vi "Main Page.vi"(8 "error in (no error)":errorcluster, 11 "Node Ptr":T1 format="%.0x") -> (0 "error out":errorcluster)   [LabVIEW 2020, in "SLSC EDS System Explorer.lvlib"]
uses:
  SLSC EDS System Explorer.lvlib
  <vilib>/NI VeriStand/Custom Device API/Custom Device Item Ref.ctl
  SLSC EDS API/JSON parsing/EDSjsonStructure.ctl
  SLSC EDS API/JSON parsing/enum.ctl
  SLSC EDS API/JSON parsing/property.ctl
  SLSC EDS API/JSON parsing/command.ctl
  SLSC EDS API/JSON parsing/scale.ctl
  SLSC EDS API/JSON parsing/physicalChannel.ctl
  SLSC EDS API/JSON parsing/register.ctl
  <vilib>/Utility/error.llb/DialogType.ctl
  <vilib>/Utility/miscctls.llb/LVStringsAndValuesArrayTypeDef_U16.ctl
  Shared/Constants.vi
  <vilib>/NI VeriStand/Custom Device API/Set Item Property (Variant).vi
  <vilib>/SLSC/Initialize Session with Devices.vi
  <vilib>/SLSC/Close Session.vi
  <vilib>/NI VeriStand/Custom Device API/Custom Device API.lvlib
  Shared/SLSC EDS Shared.lvlib
  SLSC UI API/SLSC Tree Control.lvlib
  SLSC CD API/SLSC CD System Explorer/SLSC CD System Explorer.lvlib
  SLSC CD API/SLSC CD Engine/SLSC CD Engine.lvlib
  <vilib>/SLSC/SLSC.lvlib
  Engine/SLSC EDS Engine.lvlib
  SLSC EDS API/SLSC EDS API.lvlib
panel:
  out "Custom Device State":string
  in  "Refresh page":bool
  out "SLSC Device Name":string
  out "Module Name":string
  in  "Help Button":bool
  out "Slot Number":i32
  out "CD Version":string caption="Version"
  in  "Header":cluster{"Section Name":string}={"Section Name"="SLSC EDS Custom Device"}
  in  "Name":string
  in  "SHDocVw.IWebBrowser":refnum<k7>(container)
  in  "Description":string
  in  "Modify Reset Value?":bool
  in  "I8":i8
  in  "U8":u8 format="%.0x"
  in  "I32":i32
  in  "U32":u32 format="%.0x"
  in  "U64":u64 format="%.0x"
  in  "I64":i64
  in  "DBL":dbl format="%#_16g"
  in  "Ring":u16(ring)
  in  "Add":bool
  in  "Remove":bool
  in  "Header 2":cluster{"Section Name":string}={"Section Name"="Custom Device Item Settings"}
  in  "Property tree":string[](tree)
  in  "Reservation Access":i32(ring)=3 items=["None"=0, "Read Only"=1, "Read/Write"=3]
  in  "Reservation Group":string
  in  "Loop rate":u32
  in  "Apply Reset":bool
  in  "Apply Default":bool
  # "ms"
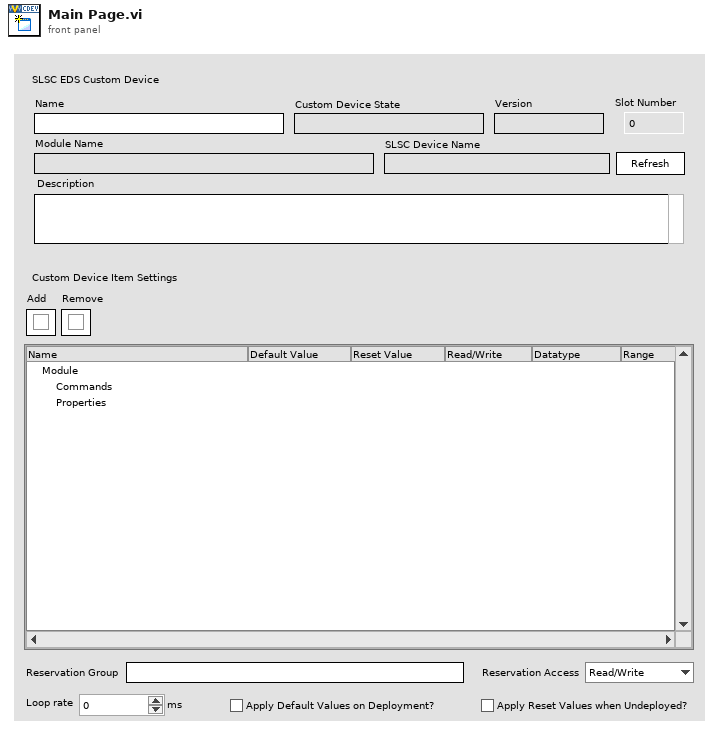
[diagram p1: front panel]
types:
  T1 = typedef "Custom Device API.lvlib/Custom Device Item Ref.ctl" = u64
  T2 = typedef "enum.ctl" = cluster{"name":string, "description-en":string, "values":cluster{"name":string, "description-en":string, "value":i32}[]}
  T3 = cluster{"Left Cell String":string, "Child Text":string[], "Child Tag":string, "Item Indent":i32, "Child Only?":bool, "Glyph Index":i32}[]
  T4 = typedef "EDSjsonStructure.ctl" = cluster{"vendorNum":u32, "vendorName":string, "vendorPrefix":string, "productNum":u32, "productName":string, "capsVersion":string, "capsSpecVersion":u32, "capsSpecOldestCompatibleVersion":u32, "enums":T2[], "properties":T5[], "commands":T6[], "scales":T7[], "physicalChannels":T8[], "registerMap":cluster{"registers":T9[]}}
  T5 = typedef "property.ctl" = cluster{"name":string, "description-en":string, "documentation-en":string, "dataType":string, "bitfield":string, "access":string, "scale":string, "value":variant, "min":variant, "max":variant, "default value":variant}
  T6 = typedef "command.ctl" = cluster{"name":string, "description-en":string, "documentation-en":string, "startBitfield":string, "waitTimeInMs":i32, "doneBitfield":string, "doneInterrupt":string, "doneTimeoutInMs":i32, "value":variant}
  T7 = typedef "scale.ctl" = cluster{"name":string, "description-en":string, "m":dbl, "b":dbl, "forwardCoeffs":dbl[], "reverseCoeffs":dbl[], "coercion":string, "table":cluster{"scaled":dbl, "unscaled":dbl}[]}
  T8 = typedef "physicalChannel.ctl" = cluster{"name":string, "description-en":string, "commands":T6[], "properties":T5[]}
  T9 = typedef "register.ctl" = cluster{"name":string, "description-en":string, "access":string, "address":u32, "size":u32, "bitfields":cluster{"name":string, "description-en":string, "offset":u32, "size":u32, "signed":bool, "strobe":bool}[]}
  T10 = typedef "LVStringsAndValuesArrayTypeDef_U16.ctl" = cluster{"String":string, "Value":u16}[]
  T11 = typedef "Custom Device API.lvlib/Custom Device Commands.ctl" = enum16{"Default", "Item renamed", "Shutdown", "Dynamic button pressed"}
  T12 = typedef "Custom Device API.lvlib/Custom Device Item Info.ctl" = cluster{"Name":string, "Is Channel":bool, "GUID":string, "Is Waveform":bool}
  T13 = typedef "DialogType.ctl" = u16
  T14 = typedef "SLSC EDS Shared.lvlib/SLSC Static Settings.ctl" = cluster{"Properties":cluster{"Boolean Properties":cluster{"property":refnum<k21>, "Value":bool, "SLSC Item":refnum<k21>, "reset value":bool}[], "Double Properties":cluster{"property":refnum<k21>, "Double Write":dbl, "SLSC Item":refnum<k21>, "Double Reset Value":dbl}[], "I32 Properties":cluster{"property":refnum<k21>, "Int32 Write":i32, "SLSC Item":refnum<k21>, "Int32 Reset Value":i32}[], "I64 Properties":cluster{"property":refnum<k21>, "Int64 Write":i64, "SLSC Item":refnum<k21>, "Int64 Reset Value":i64}[], "String Properties":cluster{"property":refnum<k21>, "String Write":string, "SLSC Item":refnum<k21>, "String Reset Value":string}[], "U32 Properties":cluster{"property":refnum<k21>, "UInt32 Write":u32, "SLSC Item":refnum<k21>, "UInt32 Reset Value":u32}[], "U64 Properties":cluster{"property":refnum<k21>, "UInt64 Write":u64, "SLSC Item":refnum<k21>, "UInt64 Reset Value":u64}[]}, "Commands":T15[], "Reset Commands":T15[], "Apply Values on Deployment":bool, "Apply Reset on Undeployment":bool, "Change Commands":T15[]}
  T15 = typedef "SLSC CD Shared.lvlib/SLSC Dynamic Channel.ctl" = cluster{"SLSC Item":string, "property":string, "Data Type":T16}
  T16 = typedef "SLSC CD Shared.lvlib/SLSC Datatype.ctl" = enum16{"Bool", "Double", "I32", "I64", "String", "U32", "U64"}
  T17 = typedef "SLSC CD Shared.lvlib/SLSC Identification.ctl" = cluster{"vendorName":string, "productNum":u32, "capsVersion":string, "capsSpecVersion":u32, "productName":string, "vendorNum":u32, "vendorPrefix":string, "capsSpecOldestCompatibleVersion":u32}
  T18 = cluster{"Left Cell String":string, "Child Text":string[], "Child Tag":string, "Item Indent":i32, "Child Only?":bool, "Glyph Index":i32}
  T19 = cluster{"name":string, "description-en":string, "value":i32}[]
  T20 = typedef "LVPoint32TypeDef.ctl" = cluster{"Horizontal":i32, "Vertical":i32}
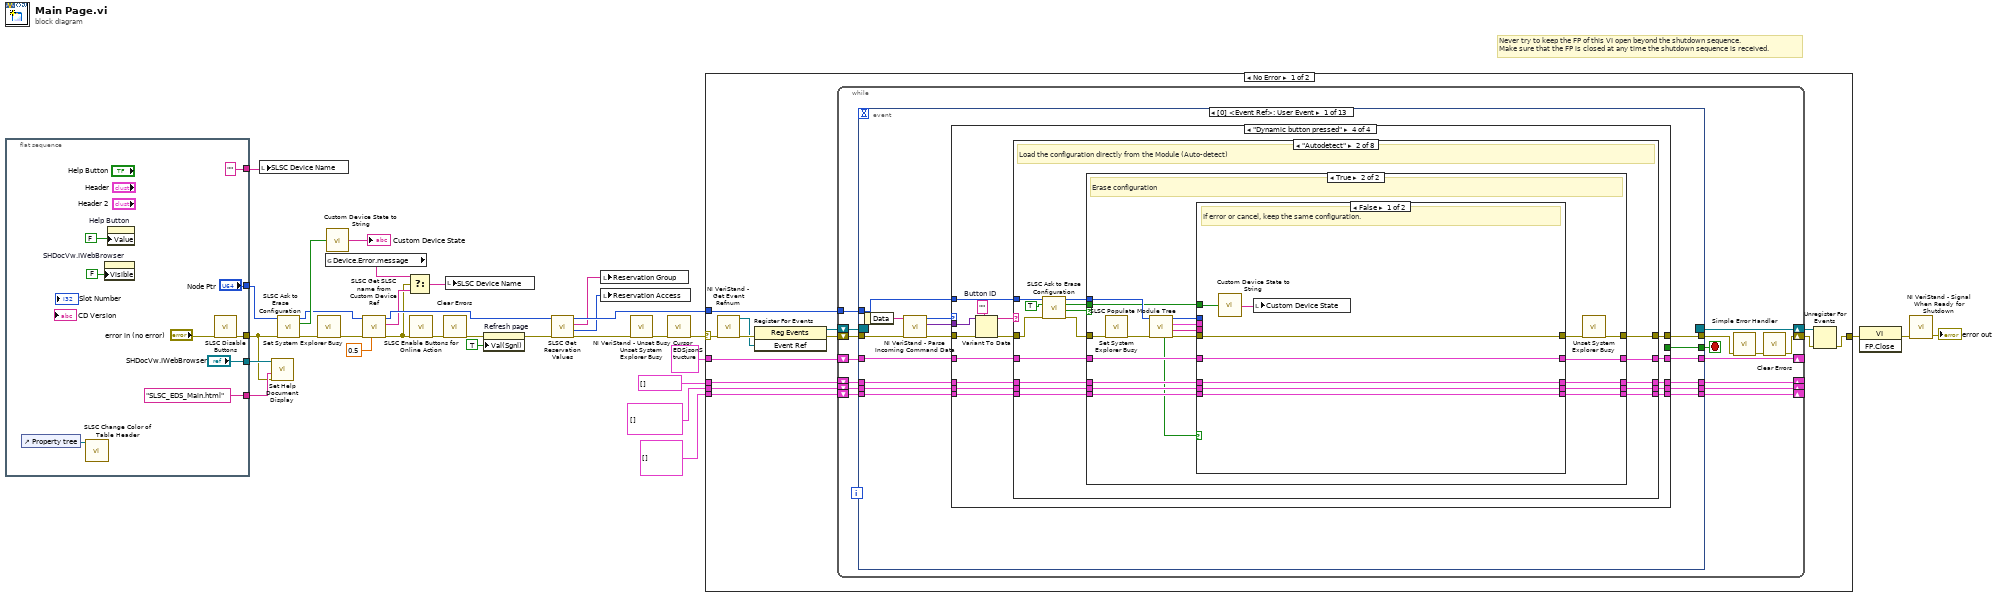
[diagram p0: block diagram]
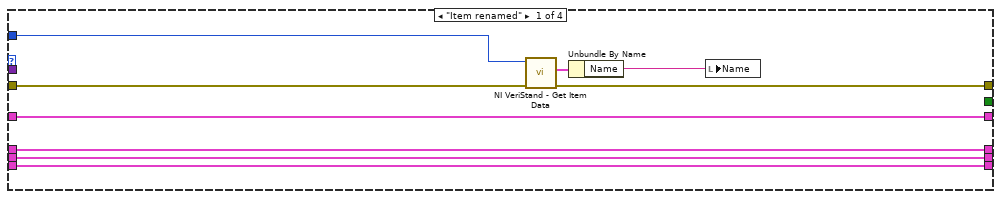
[diagram p2: hidden frame]
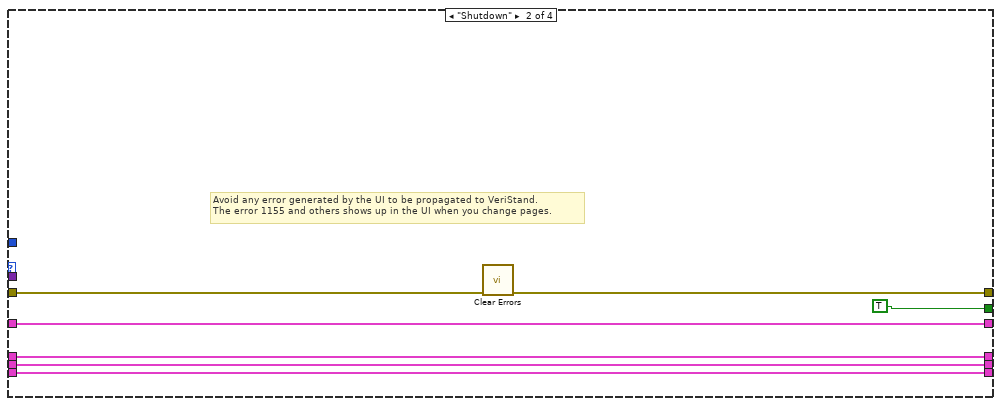
[diagram p3: hidden frame]
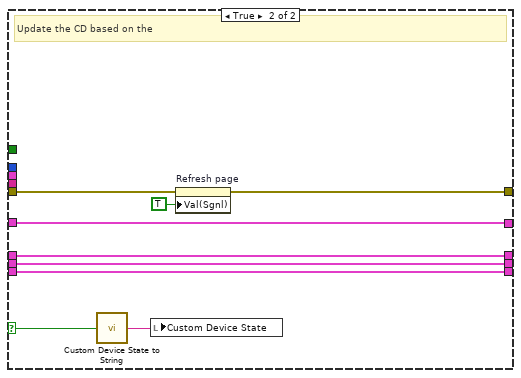
[diagram p7: hidden frame]
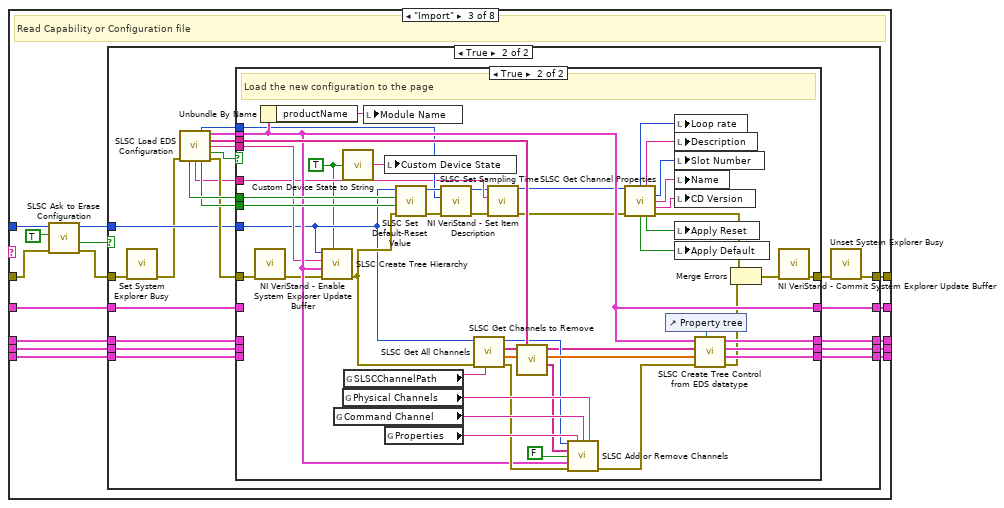
[diagram p8: hidden frame]
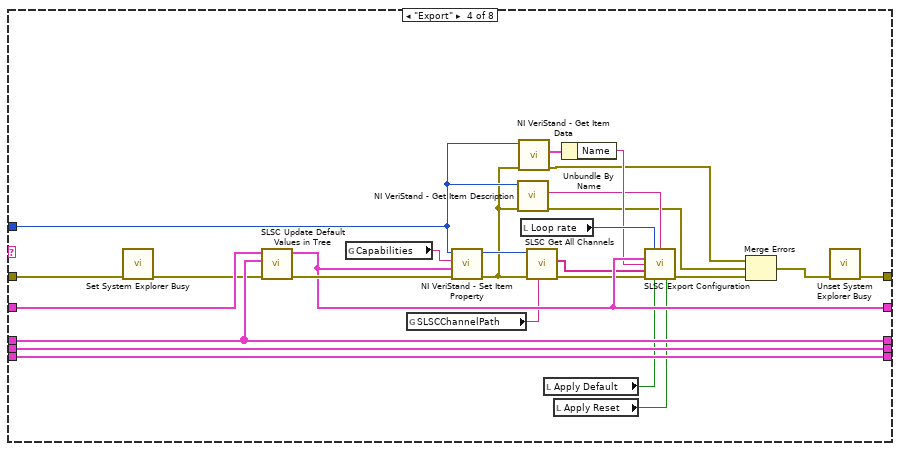
[diagram p11: hidden frame]
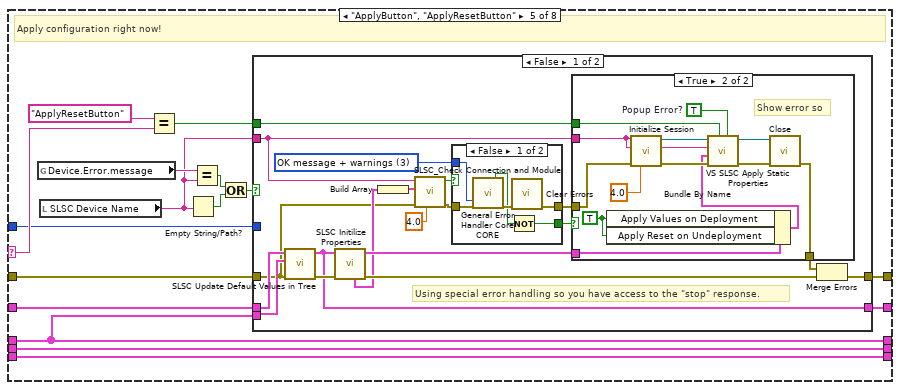
[diagram p12: hidden frame]
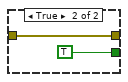
[diagram p14: hidden frame]
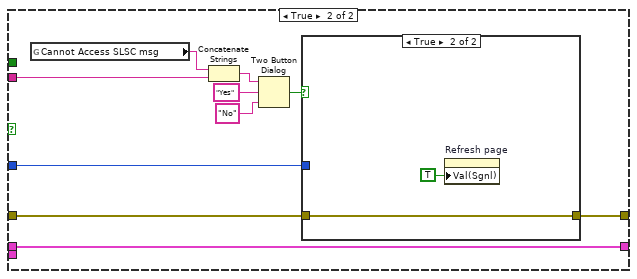
[diagram p15: hidden frame]
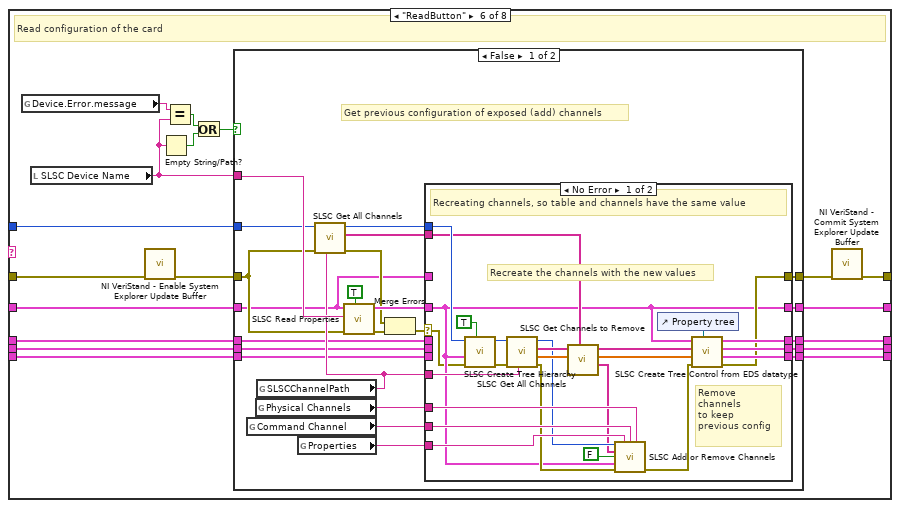
[diagram p17: hidden frame]
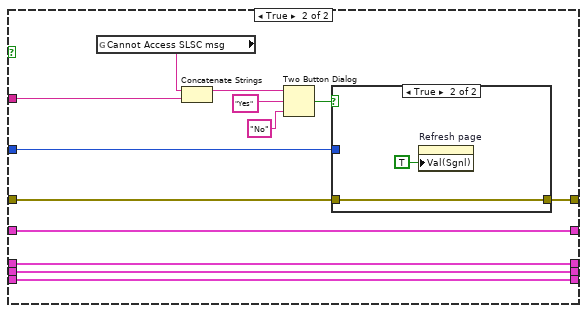
[diagram p19: hidden frame]
diagram:
  # "Never try to keep the FP of this VI open beyond the shutdown sequence.\nMake sure that the FP is closed at any time the shutdown sequence is received."
  n1 = flat-sequence {
    tunnel: ["Node Ptr"] -> w27
    tunnel: [w34] -> w28
    tunnel: ["SHDocVw.IWebBrowser"] -> w31
    tunnel: ["SLSC_EDS_Main.html" ("HTML File")] -> w30
    tunnel: ["" ("SLSC Module Name")] -> w29
    frame #0 {
      n2 = control-ref of="Property tree"() -> (w35:refnum<vi>)
      n3 = call "SLSC Change Color of Table Header.vi"("TreeControl in"=w35) -> ()  [unwired: 10 in, 1 out]
      n4 = property on="SHDocVw.IWebBrowser" class="AXCont"("Visible"=FALSE) -> ()  [unwired: 2 in, 2 out]
      n5 = property on="Help Button" class="Bool (strict)"("Value"=FALSE ("Visible")) -> ()  [unwired: 2 in, 2 out]
      n6 = call "SLSC Disable Buttons.vi"("error in (no error)"="error in (no error)") -> ("error out"=w34:errorcluster)  [unwired: 10 in]
    }
  }
  n7 = local write "SLSC Device Name"(w29) -> ()
  n8 = call "Set Help Document Display.vi"("error in (no error)"=w28, "HTML File to Load"=w30, "SHDocVw.IWebBrowser2"=w31) -> ()  [unwired: 8 in, 1 out]
  n9 = call "SLSC Ask to Erase Configuration.vi"("error in (no error)"=w28, "Device Item Ref in"=w27) -> ("error out"=w12:errorcluster, "initialized?"=w21:bool, "Item Ref out"=w10:T1)  [unwired: 6 in, 1 out]
  n10 = call "Set System Explorer Busy.vi"("error in (no error)"=w12) -> ("error out"=w11:errorcluster)  [unwired: 10 in]
  n11 = global read "Constants.vi" "Device.Error.message"() -> (w2:string)
  n12 = call "Custom Device State to String.vi"("Initialized?"=w21) -> ("Custom Device State"=→"Custom Device State":string)  [unwired: 14 in]
  n13 = call "SLSC Get SLSC name from Custom Device Ref.vi"("connect timeout"=0.5 ("connect timeout (4s)"), "error in (no error)"=w11, "Item Ref in"=w10) -> ("error out"=w4:errorcluster, "SLSC Module Name"=w5:string, "Item Ref out"=w6:T1)  [unwired: 5 in, 1 out]
  n14 = Select(t=w2, s=w4, f=w5) -> (s? t:f=w3:string)
  n15 = call "SLSC Enable Buttons for Online Action.vi"("error in (no error)"=w4) -> ("error out"=w7:errorcluster)  [unwired: 10 in]
  n16 = call <vilib>:"Clear Errors.vi"("error in (no error)"=w7) -> ("error out"=w14:errorcluster)  [unwired: 1 in, 5 out]
  n17 = local write "SLSC Device Name"(w3) -> ()
  n18 = property on="Refresh page" class="Bool (strict)"(error in=w14, "Val(Sgnl)"=TRUE ("Value (Signaling)")) -> (error out=w15:errorcluster)  [unwired: 1 in, 1 out]
  n19 = call "SLSC Get Reservation Values.vi"("Error In"=w15, "Item Ref In"=w6) -> ("Error Out"=w13:errorcluster, "Reservation Access"=w23:i32, "Reservation Group"=w24:string, "Item Ref Out"=w25:T1)  [unwired: 6 in]
  n20 = local write "Reservation Group"(w24) -> ()
  n21 = local write "Reservation Access"(w23) -> ()
  n22 = call "Unset System Explorer Busy.vi"("error in (no error)"=w13) -> ("error out"=w9:errorcluster)  [unwired: 10 in]
  n23 = call <vilib>:"NI VeriStand - Unset Busy Cursor.vi"("error in (no error)"=w9) -> ("error out"=w8:errorcluster)  [unwired: 10 in]
  n24 = case shown="No Error" w8 {
    selector: w8 -> [w47 w942]
    tunnel: [w52 w943] -> w33
    tunnel: w25 -> [w48 _]
    tunnel: T4 {"vendorNum"=0, "vendorName"="", "vendorPrefix"="", "productNum"=0, "productName"="", "capsVersion"="", "capsSpecVersion"=0, "capsSpecOldestCompatibleVersion"=1, "enums"=[], "properties"=[], "commands"=[], "scales"=[], "physicalChannels"=[], "registerMap"={"registers"=[]}} ("SLSC EDS module out") -> [w46 _]
    tunnel: T3 [] ("SLSC Output Tree") -> [w45 _]
    tunnel: T2[] [] ("Enums") -> [w44 _]
    tunnel: cluster{"name":string, string}[] [] ("Enum Strings") -> [w43 _]
    frame No Error {
      n25 = call <vilib>:"NI VeriStand - Get Event Refnum.vi"("error in (no error)"=w47) -> ("error out"=w55:errorcluster, "Event Ref"=w51:refnum<user-event>)  [unwired: 9 out]
      n26 = register-events(error in=w55, w51) -> (reference out=w49:refnum<event-registration>, error out=w50:errorcluster)  [unwired: 1 in]
      n27 = while {
        tunnel: w48 -> [w67]
        shift-right: [w65] -> w53
        shift-left: w50 -> [w70]
        shift-right: [w71] -> w54
        shift-left: w49 -> [w69]
        shift-right: [w61] -> _
        shift-left: w45 -> [w63]
        shift-right: [w59] -> _
        shift-left: w46 -> [w64]
        shift-right: [w58] -> _
        shift-left: w44 -> [w62]
        shift-right: [w57] -> _
        shift-left: w43 -> [w60]
        stop <- w68 stop-if-true
        n28 = event shown="[0] <Event Ref>: User Event" {
          selector: w69 -> [_ _ _ w802 _ _ _ _ _ _ _ _ _]
          dyn-events: [_ _ _ w802 _ _ _ _ _ _ _ _ _] -> w71
          timeout: _ -> [_ _ _ _ _ _ _ _ _ _ _ _ _]
          tunnel: w70 -> [w87 w496 w775 w795 w803 w846 w863 w870 w877 w889 w896 w898 w939]
          tunnel: [w83 _ _ _ _ _ _ _ _ _ _ _ _] -> w68
          tunnel: [w82 w496 w774 w794 w808 w813 w863 w864 w876 w888 w895 w899 w925] -> w56
          tunnel: w67 -> [w81 _ _ _ w804 w842 _ w871 w875 w887 w897 w908 w922]
          tunnel: w64 -> [w79 w495 w782 w801 w807 _ w860 w868 w878 w885 w892 w911 w931]
          tunnel: w63 -> [w78 w498 w783 w800 w810 _ w861 w872 w879 w886 w893 w916 w937]
          tunnel: w62 -> [w75 w491 w784 w797 w805 _ w858 w866 w880 w883 w890 w909 w928]
          tunnel: [w76 w498 w783 w800 w810 w827 w861 w872 w879 w886 w893 w916 w924] -> w61
          tunnel: w60 -> [w74 w492 w785 w798 w806 _ w859 w867 w881 w884 w891 w910 w929]
          tunnel: [w77 w495 w782 w801 w807 w817 w860 w868 w878 w885 w892 w911 w923] -> w59
          tunnel: [w73 w491 w784 w797 w805 w826 w858 w866 w880 w883 w890 w909 w928] -> w58
          tunnel: [w72 w492 w785 w798 w806 w825 w859 w867 w881 w884 w891 w910 w929] -> w57
          event User Event {
            n29 = event-data() -> ("Data"=w86:string)  [unwired: 1 out]
            n30 = call <vilib>:"NI VeriStand - Parse Incoming Command Data.vi"("error in (no error)"=w87, "Incoming data"=w86) -> ("error out"=w85:errorcluster, "Outgoing data"=w80:variant, "Action"=w84:T11)  [unwired: 7 out]
            n31 = case shown="\"Dynamic button pressed\"" w84 {
              tunnel: w85 -> [w96 w97 w108 w123]
              tunnel: [_ TRUE _ _] -> w83
              tunnel: [w93 w99 w108 w118] -> w82
              tunnel: w81 -> [w95 _ _ w115]
              tunnel: w80 -> [_ _ _ w122]
              tunnel: w79 -> [w91 w98 w107 w116]
              tunnel: w78 -> [w90 w102 w106 w117]
              tunnel: [w91 w98 w107 w114] -> w77
              tunnel: [w90 w102 w106 w113] -> w76
              tunnel: w75 -> [w88 w100 w104 w112]
              tunnel: w74 -> [w89 w101 w105 w111]
              tunnel: [w88 w100 w104 w110] -> w73
              tunnel: [w89 w101 w105 w109] -> w72
              frame "Item renamed" {
                n32 = call <vilib>:"NI VeriStand - Get Item Data.vi"("error in (no error)"=w96, "Item Ref in"=w95) -> ("error out"=w93:errorcluster, "Item Info"=w94:T12)  [unwired: 8 out]
                n33 = Unbundle By Name(w94) -> ("Name"=w92:string)
                n34 = local write "Name"(w92) -> ()
              }
              frame "Shutdown" {
                # "Avoid any error generated by the UI to be propagated to VeriStand.\nThe error 1155 and others shows up in the UI when you change pages."
                n35 = call <vilib>:"Clear Errors.vi"("error in (no error)"=w97) -> ("error out"=w99:errorcluster)  [unwired: 1 in, 5 out]
              }
              frame "Default", Default {
              }
              frame "Dynamic button pressed" {
                w121 = ""  # Button ID
                n36 = Variant To Data(error in=w123, type=w121, Variant=w122) -> (data=w120:string, error out=w119:errorcluster)
                n37 = case shown="\"Autodetect\"" w120 {
                  selector: w120 -> [_ _ _ _ w320 _ w467 _]
                  tunnel: w119 -> [w128 w135 w189 w301 w317 w383 w468 w484]
                  tunnel: [w128 w136 w191 w280 w316 w381 w471 w483] -> w118
                  tunnel: w117 -> [w126 w140 w195 w303 w313 w393 w465 w481]
                  tunnel: w116 -> [w127 w137 w193 w302 w321 w392 w466 w482]
                  tunnel: w115 -> [_ w134 w188 w288 w315 w391 _ _]
                  tunnel: [w127 w141 w192 w297 w314 w389 w466 w482] -> w114
                  tunnel: [w126 w142 w199 w303 w313 w388 w465 w481] -> w113
                  tunnel: w112 -> [w125 w139 w196 w298 w312 w387 w463 w479]
                  tunnel: w111 -> [w124 w138 w194 w299 w311 w386 w464 w480]
                  tunnel: [w125 w143 w198 w298 w312 w385 w463 w479] -> w110
                  tunnel: [w124 w144 w197 w299 w311 w384 w464 w480] -> w109
                  frame Default {
                  }
                  frame "Autodetect" {
                    # "Load the configuration directly from the Module (Auto-detect)"
                    n38 = call "SLSC Ask to Erase Configuration.vi"("error in (no error)"=w135, "Ask to erase?"=TRUE, "Device Item Ref in"=w134) -> ("error out"=w131:errorcluster, "Erase Data?"=w130:bool, "initialized?"=w129:bool, "Item Ref out"=w133:T1)  [unwired: 5 in]
                    n39 = case shown="True" w130 {
                      tunnel: [w147 w165] -> w144
                      tunnel: [w148 w164] -> w143
                      tunnel: [w149 w163] -> w142
                      tunnel: [w146 w162] -> w141
                      tunnel: w140 -> [w149 w160]
                      tunnel: w139 -> [w148 w159]
                      tunnel: w138 -> [w147 w158]
                      tunnel: w137 -> [w146 w157]
                      tunnel: [w145 w152] -> w136
                      tunnel: w133 -> [_ w155]
                      tunnel: w131 -> [w145 w151]
                      tunnel: w129 -> [_ w154]
                      frame False {
                        # "You decided not to erase previous configuration"
                      }
                      frame True {
                        # "Erase configuration"
                        n40 = call "Set System Explorer Busy.vi"("error in (no error)"=w151) -> ("error out"=w150:errorcluster)  [unwired: 10 in]
                        n41 = call "SLSC Populate Module Tree.vi"("error in (no error)"=w150, "Device Item Ref in"=w155) -> ("error out"=w166:errorcluster, "SLSC Module Name"=w161:string, "SLSC EDS module"=w168:T4, "Device Item Ref out"=w167:T1, "Initialized?"=w156:bool)  [unwired: 5 in]
                        n42 = case shown="False" w156 {
                          selector: w156 -> [_ w184]
                          tunnel: w168 -> [_ _]
                          tunnel: w167 -> [_ _]
                          tunnel: w166 -> [w171 w177]
                          tunnel: [w173 w179] -> w165
                          tunnel: [w174 w180] -> w164
                          tunnel: [w175 w181] -> w163
                          tunnel: [w172 w182] -> w162
                          tunnel: w161 -> [_ _]
                          tunnel: [w171 w176] -> w153
                          tunnel: w160 -> [w175 w181]
                          tunnel: w159 -> [w174 w180]
                          tunnel: w158 -> [w173 w179]
                          tunnel: w157 -> [w172 w182]
                          tunnel: w154 -> [w169 _]
                          frame False {
                            # "If error or cancel, keep the same configuration."
                            n43 = call "Custom Device State to String.vi"("Initialized?"=w169) -> ("Custom Device State"=w170:string)  [unwired: 14 in]
                            n44 = local write "Custom Device State"(w170) -> ()
                          }
                          frame True {
                            # "Update the CD based on the"
                            n45 = call "Custom Device State to String.vi"("Initialized?"=w184) -> ("Custom Device State"=w183:string)  [unwired: 14 in]
                            n46 = local write "Custom Device State"(w183) -> ()
                            n47 = property on="Refresh page" class="Bool (strict)"(error in=w177, "Val(Sgnl)"=TRUE ("Value (Signaling)")) -> (error out=w176:errorcluster)  [unwired: 1 in, 1 out]
                          }
                        }
                        n48 = call "Unset System Explorer Busy.vi"("error in (no error)"=w153) -> ("error out"=w152:errorcluster)  [unwired: 10 in]
                      }
                    }
                  }
                  frame "Import" {
                    # "Read Capability or Configuration file"
                    n49 = call "SLSC Ask to Erase Configuration.vi"("error in (no error)"=w189, "Ask to erase?"=TRUE, "Device Item Ref in"=w188) -> ("error out"=w186:errorcluster, "Erase Data?"=w185:bool, "Item Ref out"=w187:T1)  [unwired: 5 in, 1 out]
                    n50 = case shown="True" w185 {
                      tunnel: [w202 w225] -> w199
                      tunnel: [w201 w224] -> w198
                      tunnel: [w200 w223] -> w197
                      tunnel: w196 -> [w201 w222]
                      tunnel: w195 -> [w202 w215]
                      tunnel: w194 -> [w200 w214]
                      tunnel: w193 -> [w204 w213]
                      tunnel: [w204 w212] -> w192
                      tunnel: [w203 w206] -> w191
                      tunnel: w186 -> [w203 w210]
                      tunnel: w187 -> [_ w209]
                      frame False {
                        # "Decided to not overwrite previous configuration"
                      }
                      frame True {
                        n51 = call "Set System Explorer Busy.vi"("error in (no error)"=w210) -> ("error out"=w205:errorcluster)  [unwired: 10 in]
                        n52 = call "SLSC Load EDS Configuration.vi"("error in (no error)"=w205) -> ("Loop rate"=w220:u32, "SLSC EDS module out"=w226:T4, "Enable Channels"=w221:string[], "Custom Device Name"=w208:string, "Has capability?"=w216:bool, "Apply Default"=w219:bool, "Custom Device Description"=w207:string, "Apply Reset"=w218:bool, "error out"=w217:errorcluster)  [unwired: 5 in, 1 out]
                        n53 = case shown="True" w216 {
                          tunnel: w209 -> [_ w236]
                          tunnel: w226 -> [_ w251]
                          tunnel: [w231 w279] -> w225
                          tunnel: [w230 w278] -> w224
                          tunnel: [w229 w277] -> w223
                          tunnel: w222 -> [w230 _]
                          tunnel: [w228 w233] -> w211
                          tunnel: w221 -> [_ w267]
                          tunnel: w220 -> [_ w244]
                          tunnel: w219 -> [_ w262]
                          tunnel: w218 -> [_ w261]
                          tunnel: w217 -> [w228 w232]
                          tunnel: w215 -> [w231 _]
                          tunnel: w214 -> [w229 _]
                          tunnel: w213 -> [w227 _]
                          tunnel: [w227 w251] -> w212
                          tunnel: w208 -> [_ w242]
                          tunnel: w207 -> [_ w240]
                          frame False {
                            # "Error in reading the file. Don't change existent configuration."
                          }
                          frame True {
                            w234 = TRUE ("Initialized?")
                            # "Load the new configuration to the page"
                            n54 = call <vilib>:"NI VeriStand - Enable System Explorer Update Buffer.vi"("error in (no error)"=w232) -> ("error out"=w243:errorcluster)  [unwired: 10 in]
                            n55 = Unbundle By Name(w251) -> ("productName"=w263:string)
                            n56 = call "SLSC Create Tree Hierarchy.vi"("Initialized?"=w234, "error in (no error)"=w243, "SLSC EDS module"=w251, "Custom Device Name"=w242, "Item Ref in"=w236) -> ("error out"=w247:errorcluster)  [unwired: 5 in, 1 out]
                            n57 = global read "Constants.vi" "Command Channel"() -> (w272:string)
                            n58 = call "Custom Device State to String.vi"("Initialized?"=w234) -> ("Custom Device State"=w235:string)  [unwired: 14 in]
                            n59 = global read "Constants.vi" "Physical Channels"() -> (w274:string)
                            n60 = global read "Constants.vi" "SLSCChannelPath"() -> (w276:string)
                            n61 = local write "Module Name"(w263) -> ()
                            n62 = local write "Custom Device State"(w235) -> ()
                            n63 = global read "Constants.vi" "Properties"() -> (w273:string)
                            n64 = call "SLSC Set Default-Reset Value.vi"("error in (no error)"=w247, "Apply Reset"=w261, "Apply Default"=w262, "Section Ref in"=w236) -> ("error out"=w246:errorcluster, "Item Ref out"=w245:T1)  [unwired: 6 in]
                            n65 = call "SLSC Set Sampling Time.vi"("error in (no error)"=w246, "Loop rate"=w244, "Section Ref in"=w245) -> ("error out"=w241:errorcluster, "Channel Ref out"=w239:T1)  [unwired: 7 in]
                            n66 = call "SLSC Get All Channels.vi"("SLSCChannelPath"=w276, "error in (no error)"=w247, "Item Ref in"=w236) -> ("error out"=w252:errorcluster, "Channel Values"=w269:dbl[], "TreeItem Channels"=w270:string[], "Item Ref out"=w266:T1)  [unwired: 5 in]
                            n67 = call <vilib>:"NI VeriStand - Set Item Description.vi"("error in (no error)"=w241, "Description"=w240, "Item Ref in"=w239) -> ("error out"=w238:errorcluster, "Item Ref out"=w237:T1)  [unwired: 7 out]
                            n68 = call "SLSC Get Channels to Remove.vi"("Channels Created"=w267, "All Channel Values"=w269, "All Channels"=w270) -> ("Channels to be Deleted"=w265:string[], "Channel Values"=w268:dbl[], "Channels to be Added"=w264:string[])  [unwired: 6 in]
                            n69 = call "SLSC Add or Remove Channels.vi"("Section Ref in"=w266, "Properties"=w273, "Command Channel"=w272, "Physical Channels"=w274, "Property tree"=w265, "Add or Remove"=FALSE, "SLSC EDS module in"=w251, "error in (no error)"=w252) -> ("error out"=w250:errorcluster)  [unwired: 6 in, 1 out]
                            n70 = call "SLSC Get Channel Properties.vi"("Node Ptr"=w237, "error in (no error)"=w238) -> ("Loop time (ms)"=w253:u32, "Description"=w259:string, "Module Number"=w257:i32, "Name"=w260:string, "Device Version"=w256:string, "Default Value"=w255:bool, "Reset Value"=w258:bool, "error out"=w254:errorcluster)  [unwired: 5 in, 1 out]
                            n71 = control-ref of="Property tree"() -> (w275:refnum<vi>)
                            n72 = local write "Loop rate"(w253) -> ()
                            n73 = local write "Description"(w259) -> ()
                            n74 = local write "Slot Number"(w257) -> ()
                            n75 = local write "Name"(w260) -> ()
                            n76 = local write "CD Version"(w256) -> ()
                            n77 = local write "Apply Reset"(w258) -> ()
                            n78 = local write "Apply Default"(w255) -> ()
                            n79 = call "SLSC Create Tree Control from EDS datatype.vi"("Property Tree"=w275, "error in (no error)"=w250, "Channel Values"=w268, "Properties to enable"=w264, "SLSC EDS module"=w251) -> ("error out"=w249:errorcluster, "Enum Strings"=w277:cluster{"name":string, string}[], "Enums"=w278:T2[], "SLSC Output Tree"=w279:T3)  [unwired: 3 in]
                            n80 = Merge Errors(w254, w249) -> (w248:errorcluster)
                            n81 = call <vilib>:"NI VeriStand - Commit System Explorer Update Buffer.vi"("error in (no error)"=w248) -> ("error out"=w233:errorcluster)  [unwired: 10 in]
                          }
                        }
                        n82 = call "Unset System Explorer Busy.vi"("error in (no error)"=w211) -> ("error out"=w206:errorcluster)  [unwired: 10 in]
                      }
                    }
                  }
                  frame "Export" {
                    n83 = call "Set System Explorer Busy.vi"("error in (no error)"=w301) -> ("error out"=w281:errorcluster)  [unwired: 10 in]
                    n84 = call "SLSC Update Default Values in Tree.vi"("error in (no error)"=w281, "SLSC Output Tree"=w303, "SLSC EDS module in"=w302) -> ("error out"=w304:errorcluster, "SLSC EDS module out"=w297:T4)  [unwired: 7 in]
                    n85 = global read "Constants.vi" "Capabilities"() -> (w305:string)
                    n86 = global read "Constants.vi" "SLSCChannelPath"() -> (w296:string)
                    n87 = call-poly <vilib>:"NI VeriStand - Set Item Property.vi"("error in (no error)"=w304, "Value"=w297, "Property Name"=w305, "Item Ref in"=w288) -> ("error out"=w287:errorcluster, "Item Ref out"=w295:T1)  [unwired: 5 in, 1 out]
                    n88 = call <vilib>:"NI VeriStand - Get Item Description.vi"("error in (no error)"=w287, "Item Ref in"=w288) -> ("error out"=w282:errorcluster, "Description"=w285:string)  [unwired: 6 in, 2 out]
                    n89 = call <vilib>:"NI VeriStand - Get Item Data.vi"("error in (no error)"=w287, "Item Ref in"=w288) -> ("error out"=w283:errorcluster, "Item Info"=w289:T12)  [unwired: 8 out]
                    n90 = local read "Loop rate"() -> (w292:u32)
                    n91 = call "SLSC Get All Channels.vi"("SLSCChannelPath"=w296, "error in (no error)"=w287, "Item Ref in"=w295) -> ("error out"=w293:errorcluster, "TreeItem Channels"=w294:string[])  [unwired: 5 in, 2 out]
                    n92 = local read "Apply Default"() -> (w291:bool)
                    n93 = local read "Apply Reset"() -> (w290:bool)
                    n94 = Unbundle By Name(w289) -> ("Name"=w286:string)
                    n95 = call "SLSC Export Configuration.vi"("Loop rate"=w292, "Description"=w285, "SLSC EDS module in"=w297, "Custom Device Name"=w286, "Channels to Enable"=w294, "error in (no error)"=w293, "Apply Default"=w291, "Apply Reset"=w290) -> ("error out"=w300:errorcluster)  [unwired: 7 in]
                    n96 = Merge Errors(w283, w282, w300) -> (w284:errorcluster)
                    n97 = call "Unset System Explorer Busy.vi"("error in (no error)"=w284) -> ("error out"=w280:errorcluster)  [unwired: 10 in]
                  }
                  frame "ApplyButton", "ApplyResetButton" {
                    # "Apply configuration right now!"
                    n98 = global read "Constants.vi" "Device.Error.message"() -> (w309:string)
                    n99 = local read "SLSC Device Name"() -> (w307:string)
                    n100 = Equal?(x="ApplyResetButton", y=w320) -> (x = y?=w319:bool)
                    n101 = Empty String/Path?(string/path=w307) -> (empty?=w310:bool)
                    n102 = Equal?(x=w309, y=w307) -> (x = y?=w308:bool)
                    n103 = Or(x=w308, y=w310) -> (x .or. y?=w306:bool)
                    n104 = case shown="False" w306 {
                      tunnel: w313 -> [w340 _]
                      tunnel: w321 -> [w332 w366]
                      tunnel: w319 -> [w339 _]
                      tunnel: w317 -> [w327 w371]
                      tunnel: [w337 w367] -> w316
                      tunnel: w307 -> [w331 w372]
                      tunnel: w315 -> [_ w370]
                      tunnel: [w333 w366] -> w314
                      frame False {
                        w322 = T13 3 items=["no dialog", "OK message", "continue or stop message", "OK message + warnings", "continue/stop + warnings"] ("type of dialog (OK msg:1)")
                        # "Using special error handling so you have access to the \"stop\" response."
                        n105 = call "SLSC Update Default Values in Tree.vi"("error in (no error)"=w327, "SLSC Output Tree"=w340, "SLSC EDS module in"=w332) -> ("error out"=w338:errorcluster, "SLSC EDS module out"=w333:T4)  [unwired: 7 in]
                        n106 = call "SLSC Initilize Properties.vi"("error in (no error)"=w338, "Capabilities"=w333) -> ("error out"=w336:errorcluster, "Configuration Data"=w335:T14, "Identification"=w330:T17)  [unwired: 5 in, 2 out]
                        n107 = Build Array(w330) -> (w329:T17[])
                        n108 = call "SLSC_Check Connection and Module.vi"("Connect timeout (s)"=4.0 ("connect timeout (10 sec)"), "error in (no error)"=w327, "Supported Modules"=w329, "devices"=w331) -> ("error out"=w325:errorcluster, "Device Found?"=w326:bool)  [unwired: 6 in]
                        n109 = case shown="False" w326 {
                          tunnel: [w355 TRUE ("T button?")] -> w324
                          tunnel: w325 -> [w359 w361]
                          tunnel: [w360 w361] -> w323
                          tunnel: w322 -> [w357 _]
                          frame False {
                            n110 = call <vilib>:"General Error Handler Core CORE.vi"("type of dialog (OK msg:1)"=w357, "error in (no error)"=w359) -> ("stop event propagated"=w356:bool, "error out"=w358:errorcluster)  [unwired: 12 in, 4 out]
                            n111 = Not(x=w356) -> (.not. x?=w355:bool)
                            n112 = call <vilib>:"Clear Errors.vi"("error in (no error)"=w358) -> ("error out"=w360:errorcluster)  [unwired: 5 in, 1 out]
                          }
                          frame True {
                          }
                        }
                        n113 = case shown="True" w324 {
                          tunnel: w339 -> [_ w349]
                          tunnel: w335 -> [_ w347]
                          tunnel: [w341 w344] -> w334
                          tunnel: w331 -> [_ w343]
                          tunnel: w323 -> [w341 w342]
                          frame False {
                            # "Avoid messaging incorrect board.\nAnd we ask just in case the user is \nsure the board is correct, just happen\nto not match the Board number"
                          }
                          frame True {
                            w345 = TRUE ("Apply Values on Deployment")
                            w348 = TRUE  # Popup Error?
                            # "Show error so"
                            n114 = Bundle By Name(cluster=w347, "Apply Values on Deployment"=w345, "Apply Reset on Undeployment"=w345) -> (w346:T14)
                            n115 = call-poly <vilib>:"Initialize Session.vi"("devices"=w343, "error in (no error)"=w342, "connect timeout (60 sec)"=4.0 ("connect timeout (10 sec)")) -> ("session out"=w353:refnum<k21>, "error out"=w354:errorcluster)  [unwired: 11 in]
                            n116 = call "VS SLSC Apply Static Properties.vi"("Popup Error?"=w348, "Reset?"=w349, "error in (no error)"=w354, "Configuration Data"=w346, "SLSC Module Name in"=w343, "Refnum in"=w353) -> ("error out"=w351:errorcluster, "Refnum out"=w350:refnum<k21>)  [unwired: 3 in, 1 out]
                            n117 = call-poly <vilib>:"Close.vi"("session in"=w350, "error in (no error)"=w351) -> ("error out"=w344:errorcluster)  [unwired: 13 in]
                          }
                        }
                        n118 = Merge Errors(w334, w336) -> (w337:errorcluster)
                      }
                      frame True {
                        n119 = global read "Constants.vi" "Cannot Access SLSC msg"() -> (w364:string)
                        n120 = Concatenate Strings(w364, w372) -> (w369:string)
                        n121 = Two Button Dialog(message=w369, 1:"No" ("F button name (\"Cancel\")"), 2:"Yes" ("F button name (\"Cancel\")")) -> (T button?=w368:bool)
                        n122 = case shown="True" w368 {
                          tunnel: w371 -> [w373 w375]
                          tunnel: w370 -> [_ _]
                          tunnel: [w373 w375] -> w367
                          frame False {
                          }
                          frame True {
                            n123 = property on="Refresh page" class="Bool (strict)"("Val(Sgnl)"=TRUE ("Value (Signaling)")) -> ()  [unwired: 2 in, 2 out]
                          }
                        }
                      }
                    }
                  }
                  frame "ReadButton" {
                    # "Read configuration of the card"
                    n124 = global read "Constants.vi" "Device.Error.message"() -> (w378:string)
                    n125 = local read "SLSC Device Name"() -> (w377:string)
                    n126 = call <vilib>:"NI VeriStand - Enable System Explorer Update Buffer.vi"("error in (no error)"=w383) -> ("error out"=w382:errorcluster)  [unwired: 10 in]
                    n127 = Empty String/Path?(string/path=w377) -> (empty?=w390:bool)
                    n128 = Equal?(x=w378, y=w377) -> (x = y?=w376:bool)
                    n129 = Or(x=w376, y=w390) -> (x .or. y?=w379:bool)
                    n130 = case shown="False" w379 {
                      tunnel: w393 -> [w397 w452]
                      tunnel: w392 -> [w398 w453]
                      tunnel: w382 -> [w404 w458]
                      tunnel: [w401 w454] -> w380
                      tunnel: w377 -> [w416 w459]
                      tunnel: w391 -> [w411 w457]
                      tunnel: [w399 w453] -> w389
                      tunnel: [w415 w452] -> w388
                      tunnel: w387 -> [w396 w450]
                      tunnel: w386 -> [w395 w449]
                      tunnel: [w407 w450] -> w385
                      tunnel: [w406 w449] -> w384
                      frame False {
                        # "Get previous configuration of exposed (add) channels"
                        n131 = global read "Constants.vi" "Command Channel"() -> (w412:string)
                        n132 = global read "Constants.vi" "Physical Channels"() -> (w414:string)
                        n133 = global read "Constants.vi" "SLSCChannelPath"() -> (w410:string)
                        n134 = global read "Constants.vi" "Properties"() -> (w413:string)
                        n135 = call "SLSC Get All Channels.vi"("SLSCChannelPath"=w410, "error in (no error)"=w404, "Item Ref in"=w411) -> ("error out"=w402:errorcluster, "TreeItem Channels"=w408:string[], "Item Ref out"=w409:T1)  [unwired: 5 in, 1 out]
                        n136 = call "SLSC Read Properties.vi"("Default Only?"=TRUE ("Read Only?"), "error in (no error)"=w404, "SLSC Device"=w416, "SLSC EDS module in"=w398) -> ("error out"=w403:errorcluster, "SLSC EDS module out"=w405:T4)  [unwired: 6 in]
                        n137 = Merge Errors(w402, w403) -> (w400:errorcluster)
                        n138 = case shown="No Error" w400 {
                          selector: w400 -> [w417 w445]
                          tunnel: [w441 w444] -> w415
                          tunnel: w414 -> [w438 _]
                          tunnel: w413 -> [w437 _]
                          tunnel: w412 -> [w436 _]
                          tunnel: w410 -> [w430 _]
                          tunnel: w409 -> [w429 _]
                          tunnel: w408 -> [w428 _]
                          tunnel: [w423 w443] -> w407
                          tunnel: [w422 w442] -> w406
                          tunnel: w405 -> [w418 _]
                          tunnel: [w419 w445] -> w401
                          tunnel: [w418 w446] -> w399
                          tunnel: w398 -> [_ w446]
                          tunnel: w397 -> [_ w444]
                          tunnel: w396 -> [_ w443]
                          tunnel: w395 -> [_ w442]
                          frame No Error {
                            # "Remove \nchannels\nto keep \nprevious config"
                            # "Recreate the channels with the new values"
                            # "Recreating channels, so table and channels have the same value"
                            n139 = call "SLSC Create Tree Hierarchy.vi"("Initialized?"=TRUE, "error in (no error)"=w417, "SLSC EDS module"=w418, "Item Ref in"=w429) -> ("error out"=w434:errorcluster, "Parent Ref out"=w433:T1)  [unwired: 6 in]
                            n140 = call "SLSC Get All Channels.vi"("SLSCChannelPath"=w430, "error in (no error)"=w434, "Item Ref in"=w433) -> ("error out"=w421:errorcluster, "Channel Values"=w431:dbl[], "TreeItem Channels"=w432:string[], "Item Ref out"=w426:T1)  [unwired: 5 in]
                            n141 = call "SLSC Get Channels to Remove.vi"("Channels Created"=w428, "All Channel Values"=w431, "All Channels"=w432) -> ("Channels to be Deleted"=w425:string[], "Channel Values"=w427:dbl[], "Channels to be Added"=w424:string[])  [unwired: 6 in]
                            n142 = call "SLSC Add or Remove Channels.vi"("Section Ref in"=w426, "Properties"=w437, "Command Channel"=w436, "Physical Channels"=w438, "Property tree"=w425, "Add or Remove"=FALSE, "SLSC EDS module in"=w418, "error in (no error)"=w421) -> ("error out"=w420:errorcluster)  [unwired: 6 in, 1 out]
                            n143 = control-ref of="Property tree"() -> (w440:refnum<vi>)
                            n144 = call "SLSC Create Tree Control from EDS datatype.vi"("Property Tree"=w440, "error in (no error)"=w420, "Channel Values"=w427, "Properties to enable"=w424, "SLSC EDS module"=w418) -> ("error out"=w419:errorcluster, "Enum Strings"=w422:cluster{"name":string, string}[], "Enums"=w423:T2[], "SLSC Output Tree"=w441:T3)  [unwired: 3 in]
                          }
                          frame Error {
                            # "If error, don't change state and report the error (outside)"
                          }
                        }
                      }
                      frame True {
                        n145 = global read "Constants.vi" "Cannot Access SLSC msg"() -> (w448:string)
                        n146 = Concatenate Strings(w448, w459) -> (w456:string)
                        n147 = Two Button Dialog(message=w456, 1:"No" ("F button name (\"Cancel\")"), 2:"Yes" ("F button name (\"Cancel\")")) -> (T button?=w455:bool)
                        n148 = case shown="True" w455 {
                          tunnel: w458 -> [w460 w462]
                          tunnel: w457 -> [_ _]
                          tunnel: [w460 w462] -> w454
                          frame False {
                          }
                          frame True {
                            n149 = property on="Refresh page" class="Bool (strict)"("Val(Sgnl)"=TRUE ("Value (Signaling)")) -> ()  [unwired: 2 in, 2 out]
                          }
                        }
                      }
                    }
                    n150 = call <vilib>:"NI VeriStand - Commit System Explorer Update Buffer.vi"("error in (no error)"=w380) -> ("error out"=w381:errorcluster)  [unwired: 10 in]
                  }
                  frame "Diagram", "Pinout" {
                    # "Open and forget..."
                    n151 = vi-ref "SLSC Show Pinout.vi"() -> (w469:refnum<vi>)
                    n152 = property class="VI Interface Type 1"(reference=w469) -> ("Name"=w470:string)  [unwired: 1 in, 2 out]
                    n153 = Unbundle By Name(w466) -> ("vendorPrefix"=w476:string, "productNum"=w475:u32)
                    n154 = Open VI Reference(type specifier VI Refnum (for type only)=w469, vi path=w470, options=128, error in (no error)=w468) -> (vi reference=w477:refnum<vi>, error out=w473:errorcluster)  [unwired: 2 in]
                    n155 = call-by-ref "Start Asynchronous Call"(reference=w477, error in=w473, "Type"=w467, "number"=w475, "Vendor Name"=w476) -> (reference out=w474:refnum<vi>, error out=w472:errorcluster)  [unwired: 9 in]
                    n156 = Close Reference(reference=w474, error in (no error)=w472) -> (error out=w471:errorcluster)
                  }
                  frame "HelpButton" {
                    # "Show Help Page"
                    n157 = property on="SHDocVw.IWebBrowser" class="AXCont"(error in=w484) -> (error out=w485:errorcluster, "Visible"=w487:bool)  [unwired: 1 in, 1 out]
                    n158 = Not(x=w487) -> (.not. x?=w486:bool)
                    n159 = property on="SHDocVw.IWebBrowser" class="AXCont"(error in=w485, "Visible"=w486) -> (error out=w483:errorcluster)  [unwired: 1 in, 1 out]
                  }
                }
              }
            }
          }
          event "Property tree": Value Change {
            n160 = event-data() -> ()  [unwired: 2 out]
            n161 = control-ref of="Modify Reset Value?"() -> (w497:refnum<vi>)
            n162 = control-ref of="DBL"() -> (w506:refnum<vi>)
            n163 = control-ref of="I8"() -> (w504:refnum<vi>)
            n164 = control-ref of="I32"() -> (w499:refnum<vi>)
            n165 = control-ref of="I64"() -> (w500:refnum<vi>)
            n166 = control-ref of="U8"() -> (w501:refnum<vi>)
            n167 = control-ref of="U32"() -> (w502:refnum<vi>)
            n168 = control-ref of="U64"() -> (w503:refnum<vi>)
            n169 = control-ref of="Ring"() -> (w505:refnum<vi>)
            n170 = Array Size(array="Property tree") -> (size(s)=w494:i32)
            n171 = Equal To 0?(x=w494) -> (x = 0?=w489:bool)
            n172 = Not Equal?(x=w494, y=1 ("x")) -> (x != y?=w493:bool)
            n173 = case shown="False" w489 {
              tunnel: "Property tree" -> [w512 _]
              tunnel: w498 -> [w513 _]
              tunnel: w491 -> [w522 _]
              tunnel: w503 -> [w523 w764]
              tunnel: w502 -> [w529 w765]
              tunnel: w501 -> [w524 w766]
              tunnel: w500 -> [w525 w767]
              tunnel: w499 -> [w526 w768]
              tunnel: w504 -> [w527 w769]
              tunnel: w505 -> [w530 w770]
              tunnel: w506 -> [w528 w771]
              tunnel: w492 -> [w519 _]
              tunnel: "Modify Reset Value?" -> [w515 _]
              tunnel: w497 -> [w516 w762]
              tunnel: w493 -> [w514 _]
              frame False {
                # "Use the default control based on the first selection"
                # "Only allow to modify the value of 1 selection, otherwise hide control."
                n174 = Index Array(array=w512) -> (element=w521:string)  [unwired: 1 in]
                n175 = call "SLSC Search Item in Tree Control.vi"("SLSC Output Tree"=w513, "Item Tag"=w521) -> ("Item"=w520:T18)  [unwired: 10 in, 3 out]
                n176 = call "SLSC Get Items from Tree Control.vi"("Item"=w520) -> ("Value"=w511:string, "Datatype"=w508:string, "Type of Channel"=w510:string, "Reset Value"=w517:string)  [unwired: 6 in, 1 out]
                n177 = case shown="True" w514 {
                  tunnel: w513 -> [_ w539]
                  tunnel: w512 -> [_ w538]
                  tunnel: w508 -> [_ w537]
                  tunnel: w510 -> [w531 w535]
                  tunnel: [w531 w534] -> w509
                  frame False {
                  }
                  frame True {
                    n178 = for {
                      tunnel: w539 -> [w549]
                      tunnel: w538 -> [w547] mode=indexing
                      tunnel: w537 -> [w546]
                      tunnel: [w545] -> w536 mode=indexing
                      tunnel: w535 -> [w542]
                      stop <- w545 continue-if-true
                      n179 = call "SLSC Search Item in Tree Control.vi"("SLSC Output Tree"=w549, "Item Tag"=w547) -> ("Item"=w548:T18)  [unwired: 10 in, 3 out]
                      n180 = call "SLSC Get Items from Tree Control.vi"("Item"=w548) -> ("Datatype"=w540:string, "Type of Channel"=w543:string)  [unwired: 6 in, 3 out]
                      n181 = Equal?(x=w542, y=w543) -> (x = y?=w541:bool)
                      n182 = Equal?(x=w540, y=w546) -> (x = y?=w544:bool)
                      n183 = And(x=w541, y=w544) -> (x .and. y?=w545:bool)
                    }
                    n184 = And Array Elements(Boolean array=w536) -> (logical AND=w532:bool)
                    n185 = Select(t=w535, s=w532, f="Diff" ("t")) -> (s? t:f=w534:string)
                  }
                }
                n186 = Select(t=w517, s=w515, f=w511) -> (s? t:f=w518:string)
                n187 = case shown="Default" w509 {
                  tunnel: w508 -> [w563 _]
                  tunnel: w530 -> [w562 w758]
                  tunnel: w529 -> [w561 w753]
                  tunnel: w528 -> [w560 w759]
                  tunnel: w527 -> [w559 w757]
                  tunnel: w526 -> [w558 w756]
                  tunnel: w525 -> [w557 w755]
                  tunnel: w524 -> [w556 w754]
                  tunnel: w523 -> [w555 w751]
                  tunnel: w522 -> [w554 _]
                  tunnel: w518 -> [w553 _]
                  tunnel: w519 -> [w552 _]
                  tunnel: w516 -> [w551 w750]
                  tunnel: w515 -> [w550 _]
                  frame Default {
                    # "Show the type of control for Writing"
                    n188 = case shown="\"U32\", \"UInt32\"" w563 {
                      selector: w563 -> [w568 w586 w602 w618 w634 w647 w668 w686 w704 w734]
                      tunnel: w562 -> [w572 w594 w610 w626 w641 w660 w678 w695 w703 w733]
                      tunnel: w561 -> [w571 w591 w605 w622 w643 w655 w672 w689 w709 w738]
                      tunnel: w560 -> [w579 w595 w611 w627 w642 w661 w679 w688 w714 w743]
                      tunnel: w559 -> [w578 w587 w609 w625 w640 w659 w677 w694 w713 w742]
                      tunnel: w558 -> [w577 w589 w603 w620 w639 w658 w676 w693 w712 w741]
                      tunnel: w557 -> [w576 w593 w608 w624 w638 w653 w675 w692 w711 w740]
                      tunnel: w556 -> [w575 w588 w607 w619 w637 w657 w674 w691 w710 w739]
                      tunnel: w555 -> [w574 w590 w604 w621 w636 w654 w671 w687 w708 w737]
                      tunnel: w554 -> [_ _ _ _ _ _ _ _ w715 _]
                      tunnel: w553 -> [w567 w585 w601 w617 w633 w646 w667 w685 w706 w735]
                      tunnel: w552 -> [_ _ _ _ _ _ _ _ w705 _]
                      tunnel: w551 -> [w564 w583 w599 w615 w631 w649 w665 w683 w699 w729]
                      tunnel: w550 -> [_ _ _ _ _ _ _ _ _ w725]
                      frame "Bool", "Boolean" {
                        w565 = TRUE ("Visible")
                        n189 = call "SLSC Convert Items - String to Variants.vi"("Datatype"=w568, "Value"=w567) -> ("Value (DBL)"=w566:dbl)  [unwired: 10 in, 3 out]
                        n190 = Build Array(w579, w571, w578, w577, w576, w575, w574) -> (w573:refnum<vi>[])
                        n191 = for {
                          tunnel: w573 -> [w581] mode=indexing
                          n192 = property class="DigNum"(reference=w581, "Visible"=FALSE) -> ()  [unwired: 1 in, 2 out]
                        }
                        n193 = property on="Ring" class="Ring (strict)"("StringsAndValues[]"=T10 [{"String"="False", "Value"=0}, {"String"="True", "Value"=1}] ("Strings And Values []")) -> (error out=w569:errorcluster)  [unwired: 2 in, 1 out]
                        n194 = property class="Ring (strict)"(reference=w572, error in=w569, "Visible"=w565, "Value"=w566) -> ()  [unwired: 2 out]
                        n195 = property class="Bool (strict)"(reference=w564, "Visible"=w565) -> ()  [unwired: 1 in, 2 out]
                      }
                      frame "I8", "Int8" {
                        w582 = TRUE ("Visible")
                        n196 = call "SLSC Convert Items - String to Variants.vi"("Datatype"=w586, "Value"=w585) -> ("Value (DBL)"=w584:dbl)  [unwired: 10 in, 3 out]
                        n197 = Build Array(w595, w594, w588, w590, w593, w589, w591) -> (w592:refnum<vi>[])
                        n198 = for {
                          tunnel: w592 -> [w597] mode=indexing
                          n199 = property class="Num"(reference=w597, "Visible"=FALSE) -> ()  [unwired: 1 in, 2 out]
                        }
                        n200 = property class="DigNum (strict)"(reference=w587, "Visible"=w582, "Value"=w584) -> ()  [unwired: 1 in, 2 out]
                        n201 = property class="Bool (strict)"(reference=w583, "Visible"=w582) -> ()  [unwired: 1 in, 2 out]
                      }
                      frame "I32", "Int32" {
                        w598 = TRUE ("Visible")
                        n202 = call "SLSC Convert Items - String to Variants.vi"("Datatype"=w602, "Value"=w601) -> ("Value (DBL)"=w600:dbl)  [unwired: 10 in, 3 out]
                        n203 = Build Array(w611, w610, w609, w604, w608, w607, w605) -> (w606:refnum<vi>[])
                        n204 = for {
                          tunnel: w606 -> [w613] mode=indexing
                          n205 = property class="Num"(reference=w613, "Visible"=FALSE) -> ()  [unwired: 1 in, 2 out]
                        }
                        n206 = property class="DigNum (strict)"(reference=w603, "Visible"=w598, "Value"=w600) -> ()  [unwired: 1 in, 2 out]
                        n207 = property class="Bool (strict)"(reference=w599, "Visible"=w598) -> ()  [unwired: 1 in, 2 out]
                      }
                      frame "U8", "UInt8" {
                        w614 = TRUE ("Visible")
                        n208 = call "SLSC Convert Items - String to Variants.vi"("Datatype"=w618, "Value"=w617) -> ("Value (DBL)"=w616:dbl)  [unwired: 10 in, 3 out]
                        n209 = Build Array(w627, w626, w625, w621, w624, w620, w622) -> (w623:refnum<vi>[])
                        n210 = for {
                          tunnel: w623 -> [w629] mode=indexing
                          n211 = property class="Num"(reference=w629, "Visible"=FALSE) -> ()  [unwired: 1 in, 2 out]
                        }
                        n212 = property class="DigNum (strict)"(reference=w619, "Visible"=w614, "Value"=w616) -> ()  [unwired: 1 in, 2 out]
                        n213 = property class="Bool (strict)"(reference=w615, "Visible"=w614) -> ()  [unwired: 1 in, 2 out]
                      }
                      frame "U32", "UInt32" {
                        w630 = TRUE ("Visible")
                        n214 = Build Array(w642, w641, w640, w639, w638, w637, w636) -> (w635:refnum<vi>[])
                        n215 = call "SLSC Convert Items - String to Variants.vi"("Datatype"=w634, "Value"=w633) -> ("Value (DBL)"=w632:dbl)  [unwired: 10 in, 3 out]
                        n216 = for {
                          tunnel: w635 -> [w645] mode=indexing
                          n217 = property class="Num"(reference=w645, "Visible"=FALSE) -> ()  [unwired: 1 in, 2 out]
                        }
                        n218 = property class="DigNum (strict)"(reference=w643, "Visible"=w630, "Value"=w632) -> ()  [unwired: 1 in, 2 out]
                        n219 = property class="Bool (strict)"(reference=w631, "Visible"=w630) -> ()  [unwired: 1 in, 2 out]
                      }
                      frame "I64", "Int64" {
                        w648 = TRUE ("Visible")
                        n220 = call "SLSC Convert Items - String to Variants.vi"("Datatype"=w647, "Value"=w646) -> ("Value"=w652:variant)  [unwired: 10 in, 3 out]
                        n221 = Build Array(w661, w660, w659, w658, w654, w657, w655) -> (w656:refnum<vi>[])
                        n222 = for {
                          tunnel: w656 -> [w663] mode=indexing
                          n223 = property class="Num"(reference=w663, "Visible"=FALSE) -> ()  [unwired: 1 in, 2 out]
                        }
                        n224 = Variant To Data(type=i64 0, Variant=w652) -> (data=w650:i64)  [unwired: 1 in, 1 out]
                        n225 = property class="DigNum (strict)"(reference=w653, "Visible"=w648, "Value"=w650) -> ()  [unwired: 1 in, 2 out]
                        n226 = property class="Bool (strict)"(reference=w649, "Visible"=w648) -> ()  [unwired: 1 in, 2 out]
                      }
                      frame "U64", "UInt64" {
                        w664 = TRUE ("Visible")
                        n227 = call "SLSC Convert Items - String to Variants.vi"("Datatype"=w668, "Value"=w667) -> ("Value"=w666:variant)  [unwired: 10 in, 3 out]
                        n228 = Build Array(w679, w678, w677, w676, w675, w674, w672) -> (w673:refnum<vi>[])
                        n229 = for {
                          tunnel: w673 -> [w681] mode=indexing
                          n230 = property class="Num"(reference=w681, "Visible"=FALSE) -> ()  [unwired: 1 in, 2 out]
                        }
                        n231 = Variant To Data(type=u64 0, Variant=w666) -> (data=w669:u64)  [unwired: 1 in, 1 out]
                        n232 = property class="Bool (strict)"(reference=w665, "Visible"=w664) -> ()  [unwired: 1 in, 2 out]
                        n233 = property class="DigNum (strict)"(reference=w671, "Visible"=w664, "Value"=w669) -> ()  [unwired: 1 in, 2 out]
                      }
                      frame "DBL", "Double" {
                        w682 = TRUE ("Visible")
                        n234 = call "SLSC Convert Items - String to Variants.vi"("Datatype"=w686, "Value"=w685) -> ("Value (DBL)"=w684:dbl)  [unwired: 10 in, 3 out]
                        n235 = Build Array(w687, w695, w694, w693, w692, w691, w689) -> (w690:refnum<vi>[])
                        n236 = for {
                          tunnel: w690 -> [w697] mode=indexing
                          n237 = property class="Num"(reference=w697, "Visible"=FALSE) -> ()  [unwired: 1 in, 2 out]
                        }
                        n238 = property class="DigNum (strict)"(reference=w688, "Visible"=w682, "Value"=w684) -> ()  [unwired: 1 in, 2 out]
                        n239 = property class="Bool (strict)"(reference=w683, "Visible"=w682) -> ()  [unwired: 1 in, 2 out]
                      }
                      frame Default {
                        n240 = Build Array(w714, w713, w712, w711, w710, w709, w708) -> (w707:refnum<vi>[])
                        n241 = call "SLSC Search and Convert ENUM Value by Name.vi"("Enum Strings"=w705, "enums"=w715, "Value"=w706, "Datatype Name"=w704) -> ("Enum"=w701:T2, "Datatype found?"=w698:bool, "Value"=w702:i32)  [unwired: 5 in]
                        n242 = for {
                          tunnel: w707 -> [w717] mode=indexing
                          n243 = property class="DigNum"(reference=w717, "Visible"=FALSE) -> ()  [unwired: 1 in, 2 out]
                        }
                        n244 = case shown="False" w698 {
                          tunnel: w701 -> [_ w720]
                          frame False {
                            # "Datatype not found: hide all controls"
                          }
                          frame True {
                            # "Show Ring control for custom datatype"
                            n245 = Unbundle By Name(w720) -> ("values"=w719:T19)
                            n246 = for {
                              tunnel: w719 -> [w724] mode=indexing
                              tunnel: [w721] -> w718 mode=indexing
                              n247 = Unbundle(w724) -> ("name"=w723:string, "value"=w722:i32)  [unwired: 1 out]
                              n248 = Bundle("name"=w723, "value"=w722) -> (w721:cluster{"name":string, "value":i32})  [unwired: 1 in]
                            }
                            n249 = property on="Ring" class="Ring (strict)"("StringsAndValues[]"=w718) -> ()  [unwired: 2 in, 2 out]
                          }
                        }
                        n250 = property class="Ring (strict)"(reference=w703, "Visible"=w698, "Value"=w702) -> (error out=w700:errorcluster)  [unwired: 1 in, 1 out]
                        n251 = property class="Bool (strict)"(reference=w699, error in=w700, "Visible"=w698) -> ()  [unwired: 2 out]
                      }
                      frame "Command" {
                        w728 = TRUE
                        n252 = Build Array(w743, w742, w741, w740, w739, w738, w737) -> (w736:refnum<vi>[])
                        n253 = call "SLSC Command Enum Constant.vi"("Option on Reset?"=w725) -> ("Array"=w730:T2[])  [unwired: 10 in, 4 out]
                        n254 = for {
                          tunnel: w736 -> [w749] mode=indexing
                          n255 = property class="DigNum"(reference=w749, "Visible"=FALSE) -> ()  [unwired: 1 in, 2 out]
                        }
                        n256 = call "SLSC Search and Convert ENUM Value by Name.vi"("enums"=w730, "Value"=w735, "Datatype Name"=w734) -> ("Enum"=w731:T2, "Value"=w732:i32)  [unwired: 6 in, 1 out]
                        n257 = Unbundle By Name(w731) -> ("values"=w727:T19)
                        n258 = for {
                          tunnel: w727 -> [w747] mode=indexing
                          tunnel: [w744] -> w726 mode=indexing
                          n259 = Unbundle(w747) -> ("name"=w746:string, "value"=w745:i32)  [unwired: 1 out]
                          n260 = Bundle("name"=w746, "value"=w745) -> (w744:cluster{"name":string, "value":i32})  [unwired: 1 in]
                        }
                        n261 = property on="Ring" class="Ring (strict)"("StringsAndValues[]"=w726) -> ()  [unwired: 2 in, 2 out]
                        n262 = property class="Ring (strict)"(reference=w733, "Visible"=w728, "Value"=w732) -> ()  [unwired: 1 in, 2 out]
                        n263 = property class="Bool (strict)"(reference=w729, "Visible"=w728) -> ()  [unwired: 1 in, 2 out]
                      }
                    }
                  }
                  frame "Diff", "Don't Read", "Multi " {
                    # "Remove the Control Change"
                    n264 = Build Array(w759, w758, w757, w756, w755, w754, w753, w751, w750) -> (w752:refnum<vi>[])
                    n265 = for {
                      tunnel: w752 -> [w761] mode=indexing
                      n266 = property class="Ctl"(reference=w761, "Visible"=FALSE) -> ()  [unwired: 1 in, 2 out]
                    }
                  }
                }
              }
              frame True {
                n267 = Build Array(w771, w770, w769, w768, w767, w766, w765, w764, w762) -> (w763:refnum<vi>[])
                n268 = for {
                  tunnel: w763 -> [w773] mode=indexing
                  n269 = property class="Ctl"(reference=w773, "Visible"=FALSE) -> ()  [unwired: 1 in, 2 out]
                }
              }
            }
          }
          event "Modify Reset Value?": Value Change {
            n270 = event-data() -> ("NewVal"=w777:bool)  [unwired: 6 out]
            n271 = control-ref of="Property tree"() -> (w778:refnum<vi>)
            n272 = Select(t=2 ("Active Cell:Active Column Number"), s=w777, f=1 ("Active Cell:Active Column Number")) -> (s? t:f=w776:i32)
            n273 = call "SLSC Change Color of Table Header.vi"("error in (no error)"=w775, "Active Cell:Active Column Number"=w776, "TreeControl in"=w778) -> ("error out"=w774:errorcluster)  [unwired: 8 in]
            n274 = local read "Property tree"() -> (w781:string[])
            n275 = property on="Property tree" class="Tree (strict)"("Val(Sgnl)"=w781) -> ()  [unwired: 2 in, 2 out]
          }
          event "Property tree": Mouse Down {
            w788 = 2 ("upper limit")
            # "-3 means no highlilght"
            # "Highlight the Default Value\nand the Reset Value only"
            n276 = event-data() -> ("Coords"=w799:T20)  [unwired: 1 out]
            n277 = invoke on="Property tree" class="Tree (strict)" method="Point To Row Column"("Point"=w799) -> ("Col"=w787:i32)  [unwired: 7 in, 7 out]
            n278 = In Range and Coerce(upper limit=w788, x=w787, lower limit=1) -> (coerced(x)=w791:i32, In Range?=w792:bool)
            n279 = Equal?(x=w787, y=w788) -> (x = y?=w786:bool)
            n280 = local write "Modify Reset Value?"(w786) -> ()
            n281 = Select(t=w791, s=w792, f=-3) -> (s? t:f=w789:i32)
            n282 = control-ref of="Property tree"() -> (w796:refnum<vi>)
            n283 = call "SLSC Change Color of Table Header.vi"("error in (no error)"=w795, "Active Cell:Active Column Number"=w789, "TreeControl in"=w796) -> ("error out"=w794:errorcluster)  [unwired: 8 in]
          }
          event "Loop rate": Value Change {
            n284 = event-data() -> ()  [unwired: 2 out]
            n285 = call "SLSC Set Sampling Time.vi"("error in (no error)"=w803, "Loop rate"="Loop rate", "Section Ref in"=w804) -> ("error out"=w808:errorcluster)  [unwired: 7 in, 1 out]
          }
          event "Refresh page": Value Change {
            n286 = event-data() -> ()  [unwired: 7 out]
            n287 = call "Set System Explorer Busy.vi"("error in (no error)"=w846) -> ("error out"=w819:errorcluster)  [unwired: 10 in]
            n288 = global read "Constants.vi" "Capabilities"() -> (w843:string)
            n289 = call "SLSC Get Capabilities from Custom Device.vi"("Property Name"=w843, "error in (no error)"=w819, "Device Item Ref in"=w842) -> ("error out"=w824:errorcluster, "data"=w811:T4, "Item Ref out"=w836:T1)  [unwired: 3 in, 3 out]
            n290 = First Call?() -> (First Call?: T/F=w812:bool)
            n291 = case shown="False" w812 {
              tunnel: [w853 w857] -> w845
              tunnel: w842 -> [w854 _]
              tunnel: w819 -> [w856 w857]
              frame False {
                n292 = global read "Constants.vi" "Device.Error.message"() -> (w849:string)
                n293 = call "SLSC Disable Buttons.vi"("error in (no error)"=w856) -> ("error out"=w855:errorcluster)  [unwired: 10 in]
                n294 = call "SLSC Get SLSC name from Custom Device Ref.vi"("connect timeout"=4.0, "error in (no error)"=w855, "Item Ref in"=w854) -> ("error out"=w851:errorcluster, "SLSC Module Name"=w850:string)  [unwired: 5 in, 2 out]
                n295 = Select(t=w849, s=w851, f=w850) -> (s? t:f=→"SLSC Device Name":string)
                n296 = call "SLSC Enable Buttons for Online Action.vi"("error in (no error)"=w851) -> ("error out"=w853:errorcluster)  [unwired: 10 in]
              }
              frame True {
              }
            }
            n297 = global read "Constants.vi" "SLSCChannelPath"() -> (w841:string)
            n298 = call "SLSC Get All Channels.vi"("SLSCChannelPath"=w841, "error in (no error)"=w824, "Item Ref in"=w836) -> ("error out"=w838:errorcluster, "Channel Values"=w840:dbl[], "TreeItem Channels"=w839:string[], "Item Ref out"=w828:T1)  [unwired: 5 in]
            n299 = control-ref of="Property tree"() -> (w837:refnum<vi>)
            n300 = call "SLSC Create Tree Control from EDS datatype.vi"("Property Tree"=w837, "error in (no error)"=w838, "Channel Values"=w840, "Properties to enable"=w839, "SLSC EDS module"=w811) -> ("error out"=w823:errorcluster, "Enum Strings"=w825:cluster{"name":string, string}[], "Enums"=w826:T2[], "SLSC Output Tree"=w827:T3)  [unwired: 3 in]
            n301 = call "SLSC Update Default Values in Tree.vi"("error in (no error)"=w823, "SLSC Output Tree"=w827, "SLSC EDS module in"=w811) -> ("error out"=w822:errorcluster, "SLSC EDS module out"=w817:T4)  [unwired: 7 in]
            n302 = call "SLSC Get Channel Properties.vi"("Node Ptr"=w828, "error in (no error)"=w822) -> ("Loop time (ms)"=w835:u32, "Description"=w833:string, "Module Number"=w830:i32, "Name"=w834:string, "Device Version"=w829:string, "Default Value"=w831:bool, "Reset Value"=w832:bool, "error out"=w820:errorcluster)  [unwired: 5 in, 1 out]
            n303 = local write "Loop rate"(w835) -> ()
            n304 = local write "Description"(w833) -> ()
            n305 = local write "Slot Number"(w830) -> ()
            n306 = local write "Name"(w834) -> ()
            n307 = local write "CD Version"(w829) -> ()
            n308 = local write "Apply Reset"(w832) -> ()
            n309 = local write "Apply Default"(w831) -> ()
            n310 = Merge Errors(w845, w820) -> (w821:errorcluster)
            n311 = call <vilib>:"Simple Error Handler.vi"("error in (no error)"=w821) -> ("error out"=w847:errorcluster)  [unwired: 1 in, 7 out]
            n312 = call <vilib>:"Clear Errors.vi"("error in (no error)"=w847) -> ("error out"=w844:errorcluster)  [unwired: 1 in, 5 out]
            n313 = Unbundle By Name(w817) -> ("productName"=→"Module Name":string)
            n314 = call "SLSC Enable Buttons.vi"("error in (no error)"=w844, "data"=w817) -> ("error out"=w818:errorcluster)  [unwired: 9 in]
            n315 = call "Unset System Explorer Busy.vi"("error in (no error)"=w818) -> ("error out"=w815:errorcluster)  [unwired: 10 in]
            n316 = property on="Refresh page" class="Bool (strict)"(error in=w815, "Value"=FALSE ("Refresh page")) -> (error out=w813:errorcluster)  [unwired: 1 in, 1 out]
          }
          event "Help Button": Value Change {
            n317 = event-data() -> ("NewVal"=w862:bool)  [unwired: 1 out]
            n318 = property on="SHDocVw.IWebBrowser" class="AXCont"("Visible"=w862) -> ()  [unwired: 2 in, 2 out]
          }
          event "Apply Reset", "Apply Default": Value Change {
            n319 = event-data() -> ()  [unwired: 7 out]
            n320 = call "SLSC Set Default-Reset Value.vi"("error in (no error)"=w870, "Apply Reset"="Apply Reset", "Apply Default"="Apply Default", "Section Ref in"=w871) -> ("error out"=w864:errorcluster)  [unwired: 6 in, 1 out]
          }
          event "Reservation Group", "Reservation Access": Value Change {
            n321 = event-data() -> ()  [unwired: 7 out]
            n322 = call "SLSC Set Reservation Values.vi"("Error In"=w877, "Reservation Access"="Reservation Access", "Reservation Group"="Reservation Group", "Item Ref In"=w875) -> ("Error Out"=w876:errorcluster)  [unwired: 6 in, 1 out]
          }
          event "Name": Value Change {
            n323 = event-data() -> ()  [unwired: 2 out]
            n324 = call <vilib>:"NI VeriStand - Rename Custom Device Item.vi"("error in (no error)"=w889, "New Name"="Name", "Item Ref in"=w887) -> ("error out"=w888:errorcluster)  [unwired: 1 in, 7 out]
          }
          event "Description": Value Change {
            n325 = event-data() -> ()  [unwired: 2 out]
            n326 = call <vilib>:"NI VeriStand - Set Item Description.vi"("error in (no error)"=w896, "Description"="Description", "Item Ref in"=w897) -> ("error out"=w895:errorcluster)  [unwired: 8 out]
          }
          event "Remove", "Add": Value Change {
            # "Remove non-critical error. Keep pop-up\nin case you need to debug."
            # "Need to update\nicons in the controls"
            n327 = event-data() -> ()  [unwired: 2 out]
            n328 = global read "Constants.vi" "Command Channel"() -> (w913:string)
            n329 = local read "Property tree"() -> (w900:string[])
            n330 = global read "Constants.vi" "Physical Channels"() -> (w912:string)
            n331 = global read "Constants.vi" "Properties"() -> (w914:string)
            n332 = call "SLSC Add or Remove Channels.vi"("Section Ref in"=w908, "Properties"=w914, "Command Channel"=w913, "Physical Channels"=w912, "Property tree"=w900, "Add or Remove"="Add", "SLSC EDS module in"=w911, "error in (no error)"=w898, "Enums"=w909) -> ("Section Ref out"=w906:T1, "error out"=w907:errorcluster)  [unwired: 5 in]
            n333 = control-ref of="Property tree"() -> (w902:refnum<vi>)
            n334 = global read "Constants.vi" "SLSCChannelPath"() -> (w901:string)
            n335 = call "SLSC Refresh Tree Control.vi"("SLSCChannelPath"=w901, "Update Only?"=TRUE, "enums"=w909, "TreeControl in"=w902, "error in (no error)"=w907, "SLSC Output Tree"=w916, "Item Ref in"=w906) -> ("error out"=w904:errorcluster)  [unwired: 3 in, 1 out]
            n336 = disable-structure shown="Enabled" {
              disable-tunnel: w904 -> [w918 w919]
              disable-tunnel: [w917 w919] -> w903
              frame Disabled {
                n337 = call <vilib>:"Simple Error Handler.vi"("error in (no error)"=w918) -> ("error out"=w917:errorcluster)  [unwired: 4 in, 4 out]
              }
              frame Enabled {
              }
            }
            n338 = flat-sequence {
              tunnel: w907 -> [w920]
              tunnel: [w920] -> w899
              frame #0 {
                w921 = FALSE ("Remove")
                n339 = local write "Remove"(w921) -> ()
                n340 = local write "Add"(w921) -> ()
              }
            }
            n341 = call <vilib>:"Clear Errors.vi"("error in (no error)"=w903) -> ()  [unwired: 1 in, 6 out]
          }
          event "Ring", "I64", "U64", "U32", "I32", "U8", "I8", "DBL": Value Change {
            n342 = event-data() -> ("NewVal"=w934:variant)  [unwired: 1 out]
            n343 = global read "Constants.vi" "Command Channel"() -> (w932:string)
            n344 = local read "Property tree"() -> (w936:string[])
            n345 = control-ref of="Property tree"() -> (w935:refnum<vi>)
            n346 = global read "Constants.vi" "Properties"() -> (w933:string)
            n347 = local read "Modify Reset Value?"() -> (w938:bool)
            n348 = call "SLSC Update Values in Tree Control.vi"("Section Ref in"=w922, "TreeControl in"=w935, "Properties"=w933, "Command Channel"=w932, "Property tree in"=w936, "NewVal"=w934, "SLSC Output Tree"=w937, "error in (no error)"=w939, "Enums"=w928, "Enum Strings"=w929, "Modify Reset Value?"=w938) -> ("SLSC Output Tree Out"=w924:T3, "error out"=w930:errorcluster)  [unwired: 3 in]
            n349 = global read "Constants.vi" "Capabilities"() -> (w927:string)
            n350 = call "SLSC Update Default Values in Tree.vi"("error in (no error)"=w930, "SLSC Output Tree"=w924, "SLSC EDS module in"=w931) -> ("error out"=w926:errorcluster, "SLSC EDS module out"=w923:T4)  [unwired: 7 in]
            n351 = call-poly <vilib>:"NI VeriStand - Set Item Property.vi"("error in (no error)"=w926, "Value"=w923, "Property Name"=w927, "Item Ref in"=w922) -> ("error out"=w925:errorcluster)  [unwired: 5 in, 2 out]
          }
        }
        n352 = call <vilib>:"Simple Error Handler.vi"("error in (no error)"=w56) -> ("error out"=w66:errorcluster)  [unwired: 1 in, 7 out]
        n353 = call <vilib>:"Clear Errors.vi"("error in (no error)"=w66) -> ("error out"=w65:errorcluster)  [unwired: 1 in, 5 out]
      }
      n354 = Unregister For Events(event registration refnum=w54, error in=w53) -> (error out=w52:errorcluster)
    }
    frame Error {
      # "#Todo: Removing errors that\ncould happen if you change\nfrom one page to another. This \nerror can make the VS 2017 driver to break. \nBut this is just a workaround... maybe we \nshould invest more time to understand why\nthis happen and how to fix it."
      n355 = call <vilib>:"Clear Errors.vi"("error in (no error)"=w942, "specific error code to clear (0: all)"=1055) -> ("error out"=w941:errorcluster)  [unwired: 4 in, 1 out]
      n356 = call <vilib>:"Simple Error Handler.vi"("error in (no error)"=w941) -> ("error out"=w944:errorcluster)  [unwired: 1 in, 7 out]
      n357 = call <vilib>:"Clear Errors.vi"("error in (no error)"=w944) -> ("error out"=w943:errorcluster)  [unwired: 1 in, 5 out]
    }
  }
  n358 = invoke class="VI" method="FP.Close"(error in=w33) -> (error out=w32:errorcluster)  [unwired: 2 in, 2 out]
  n359 = call <vilib>:"NI VeriStand - Signal When Ready for Shutdown.vi"("error in (no error)"=w32) -> ("error out"=→"error out":errorcluster)  [unwired: 10 out]
